vi "AutoLoadRoutines.vi"(1 "Reload Routines":bool, 2 "MotionPlanningNotifiers":T1, 3 "Auto Routines Storage Directory":path=path "/home/lvuser/AutoRoutines") -> (0 "Auto Routines":T2)   [LabVIEW 2017]
uses:
  TypeDef/AutoRoutines.ctl
  TypeDef/AutoRoutineSet.ctl
  TypeDefs/RobotComponents/MotionPlanningNotifiers.ctl
  PathPlannerSupport/TypeDefs/DrivePlanRequest.ctl
  TypeDef/AutoWaypointType.ctl
  Pathfinder/Pathfinder-LabVIEW/Pathfinder-Lib/VIs/Waypoint.ctl
  PathPlannerSupport/TypeDefs/DrivePlanResponse.ctl
  Pathfinder/Pathfinder-LabVIEW/Pathfinder-Lib/VIs/Segment.ctl
  Implements/Arm/TypeDefs/ArmPlanRequest.ctl
  Implements/Arm/TypeDefs/ArmTargetPosition.ctl
  Implements/Arm/TypeDefs/ArmPlanResponse.ctl
  General/MotionProfiling/TypeDefs/TrajectoryPoint.ctl
  <vilib>/Rock Robotics/WPI/ThirdParty/Phoenix-LabVIEW/Motor Controller/Controls/CTRE_Phoenix_MotorControl_TrajectoryPointTimeDur.ctl
  TypeDef/AutoStartingPositions.ctl
  TypeDef/AutoStep.ctl
  Implements/TypeDefs/IntakeState.ctl
  e61514f7-18c3-42f3-b2a8-fda8a5312ef7.vi
  55916f22-7f41-4e59-abc4-9fcd15d20e92.vi
  058e71e0-aaa7-4a66-86c1-b77b5f723853.vi
  <vilib>/Utility/file.llb/Read Delimited Spreadsheet (DBL).vi
  Pathfinder/Pathfinder-LabVIEW/Pathfinder-Lib/Pathfinder.lvlib
panel:
  in  "BackgroundFilePath":path=path "/home/lvuser/AutoPathImages/Background.png"
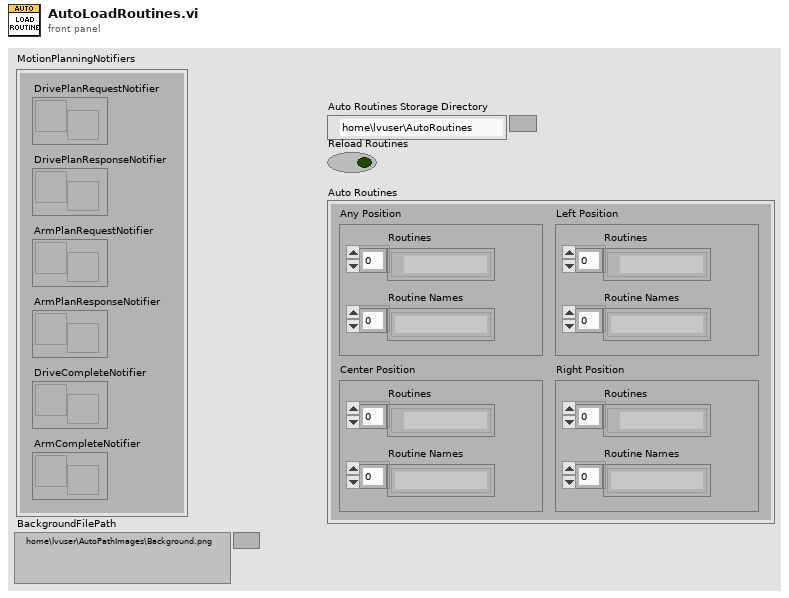
[diagram p1: front panel]
types:
  T1 = typedef "MotionPlanningNotifiers.ctl" = cluster{"DrivePlanRequestNotifier":refnum<notifier>, "DrivePlanResponseNotifier":refnum<notifier>, "ArmPlanRequestNotifier":refnum<notifier>, "ArmPlanResponseNotifier":refnum<notifier>, "DriveCompleteNotifier":refnum<notifier>, "ArmCompleteNotifier":refnum<notifier>}
  T2 = typedef "AutoRoutines.ctl" = cluster{"Any Position":T3, "Left Position":T3, "Center Position":T3, "Right Position":T3}
  T3 = typedef "AutoRoutineSet.ctl" = cluster{"Routine Names":string[], "Routines":path[]}
  T4 = typedef "AutoStartingPositions.ctl" = enum16{"Any", "Left", "Center", "Right"}
  T5 = typedef "ArmTargetPosition.ctl" = enum16{"Hold", "Switch", "Scale Low", "Scale High", "Climb", "Back Place"}
  T6 = typedef "IntakeState.ctl" = enum16{"Stop", "Forward", "Reverse", "Forward Open"}
  T7 = typedef "AutoWaypointType.ctl" = enum16{"Pathfinder Endpoint", "Pathfinder Waypoint", "Zero-Radius Turn Endpoint", "Stationary", "Vision Assist Endpoint", "Stop"}
  T8 = typedef "AutoStep.ctl" = cluster{"Waypoint Type":T7, "Waypoint":T9, "WaitTime (ms)":u16, "ArmPosition":T5, "IntakeState":T6, "Claw Open":bool, "ArmOffsetTime (ms)":u16, "ClawReleaseTime (ms)":i32}
  T9 = typedef "Pathfinder.lvlib/Waypoint.ctl" = cluster{"x":dbl, "y":dbl, "angle":dbl}
  T10 = typedef "AutoPreProcessedStep.ctl" = cluster{"DrivePath":T11, "ArmPath":T13, "Waypoint Type":T7, "WaitTime (ms)":u16, "ArmPosition":T5, "IntakeState":T6, "Claw Open":bool, "ArmOffsetTime (ms)":u16, "ClawReleaseTime (ms)":i32}
  T11 = typedef "DrivePlanResponse.ctl" = cluster{"LeftDriveTrajectory":T12[], "RightDriveTrajectory":T12[], "PlanTime (ms)":u32, "Execute":bool}
  T12 = typedef "Pathfinder.lvlib/Segment.ctl" = cluster{"dt":dbl, "x":dbl, "y":dbl, "position":dbl, "velocity":dbl, "acceleration":dbl, "jerk":dbl, "heading":dbl}
  T13 = typedef "ArmPlanResponse.ctl" = cluster{"RotateTrajectory":T14[], "ExtendTrajectory":T14[], "PlanTime (ms)":u32, "Execute":bool}
  T14 = typedef "TrajectoryPoint.ctl" = cluster{"Position ":dbl, "Velocity ":dbl, "Time (ms)":T15, "Last Point":bool}
  T15 = typedef "CTRE_Phoenix_MotorControl_TrajectoryPointTimeDur.ctl" = i32
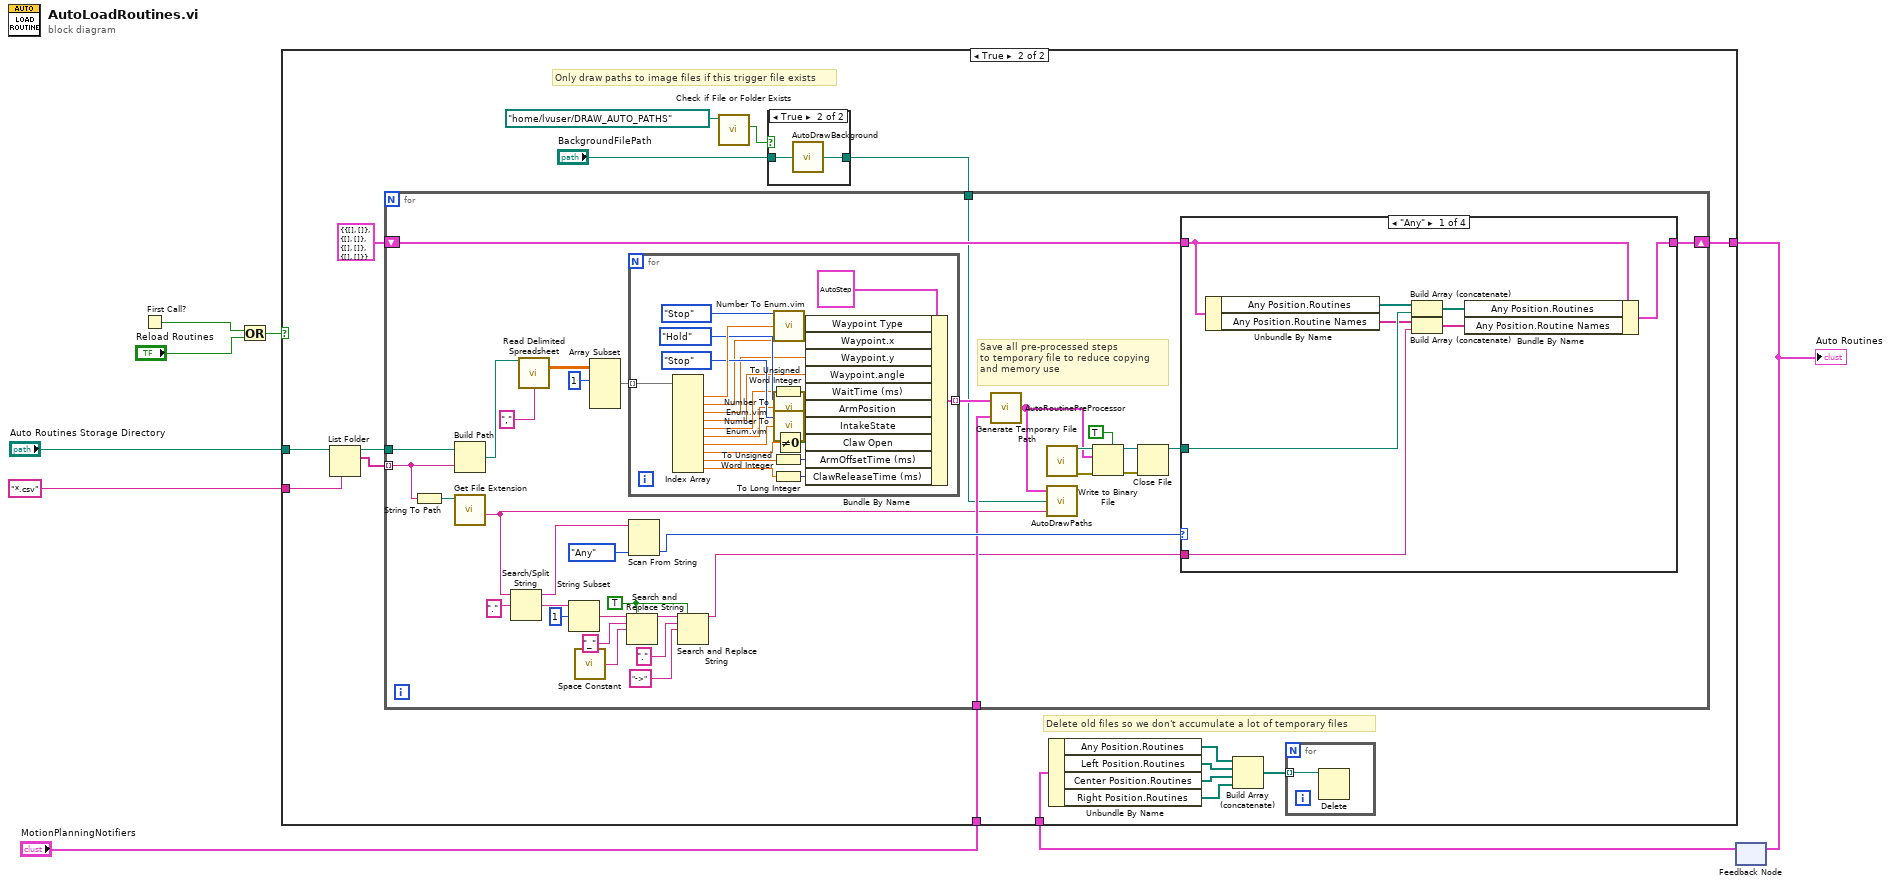
[diagram p0: block diagram]
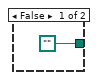
[diagram p3: hidden frame]
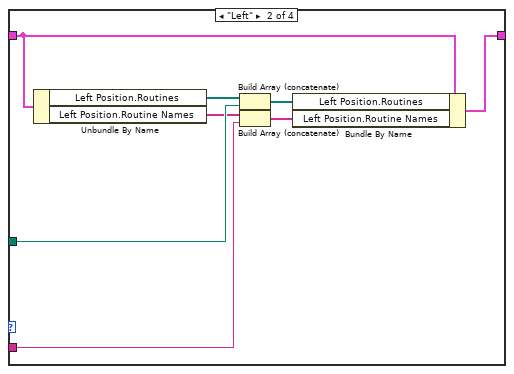
[diagram p4: hidden frame]
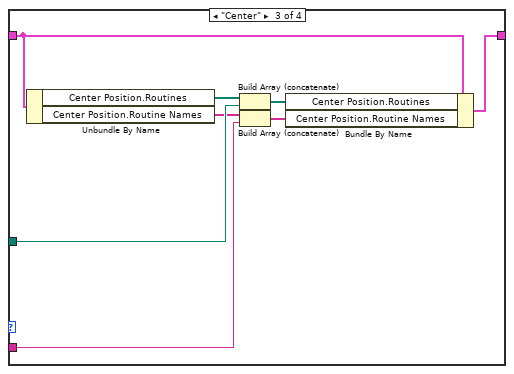
[diagram p5: hidden frame]
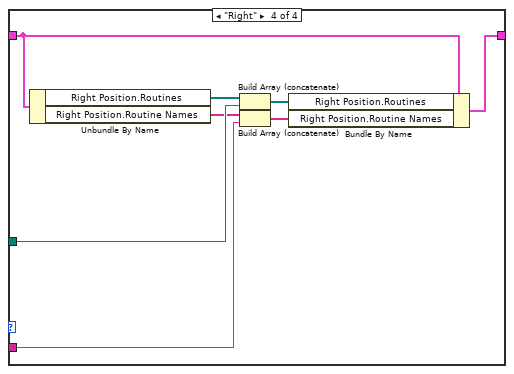
[diagram p6: hidden frame]
diagram:
  n1 = First Call?() -> (First Call?: T/F=w4:bool)
  n2 = Or(x=w4, y="Reload Routines") -> (x .or. y?=w6:bool)
  n3 = feedback #1() -> (w3:T2)  [unwired: 1 in]
  n4 = case shown="True" w6 {
    tunnel: "Auto Routines Storage Directory" -> [_ w26]
    tunnel: "*.csv" ("pattern") -> [_ w25]
    tunnel: [w9 w21] -> w2
    tunnel: w3 -> [w9 w19]
    tunnel: "MotionPlanningNotifiers" -> [_ w20]
    frame False {
    }
    frame True {
      # "Only draw paths to image files if this trigger file exists"
      # "Delete old files so we don't accumulate a lot of temporary files"
      n5 = List Folder(path=w26, pattern=w25) -> (path out=w24:path, filenames=w23:string[])  [unwired: 2 in, 2 out]
      n6 = call <vilib>:"Check if File or Folder Exists.vi"("path"=path "/home/lvuser/DRAW_AUTO_PATHS") -> ("file or folder exists?"=w11:bool)  [unwired: 8 in, 2 out]
      n7 = case shown="True" w11 {
        tunnel: "BackgroundFilePath" -> [_ w29]
        tunnel: [path "" w28] -> w12
        frame False {
        }
        frame True {
          n8 = call "AutoDrawBackground.vi"("File Path"=w29) -> ("File Path Out"=w28:path)
        }
      }
      n9 = for {
        tunnel: w24 -> [w62]
        tunnel: w23 -> [w43] mode=indexing
        shift-right: [w45] -> w21
        shift-left: T2 {"Any Position"={"Routine Names"=[], "Routines"=[]}, "Left Position"={"Routine Names"=[], "Routines"=[]}, "Center Position"={"Routine Names"=[], "Routines"=[]}, "Right Position"={"Routine Names"=[], "Routines"=[]}} ("Auto Routine") -> [w46]
        tunnel: w20 -> [w41]
        tunnel: w12 -> [w31]
        w53 = TRUE ("replace all? (F)")
        # "Save all pre-processed steps\nto temporary file to reduce copying\nand memory use"
        n10 = String To Path(string=w43) -> (path=w44:path)
        n11 = Build Path(base path=w62, name or relative path=w43) -> (appended path=w64:path)
        n12 = call <vilib>:"Get File Extension.vi"("file"=w44) -> ("filename without extension"=w32:string)  [unwired: 6 in, 4 out]
        n13 = Search/Split String(string=w32, search string/char (-)=".") -> (substring before match=w49:string, match + rest of string=w61:string)  [unwired: 1 in, 1 out]
        n14 = call-poly <vilib>:"Read Delimited Spreadsheet.vi"("file path (dialog if empty)"=w64, "delimiter (\\t)"="," ("delimiter (\\t)")) -> ("all rows"=w52:dbl[][])  [unwired: 8 in, 5 out]
        n15 = String Subset(string=w61, offset (0)=1) -> (substring=w59:string)  [unwired: 1 in]
        n16 = call <vilib>:"Space Constant.vi"() -> ("String"=w57:string)
        n17 = Array Subset(array=w52, index (row)=1 ("index")) -> (w50:dbl[][])  [unwired: 3 in]
        n18 = Search and Replace String(replace all?=w53, input string=w59, search string="_", replace string=w57) -> (result string=w56:string)  [unwired: 4 in, 3 out]
        n19 = for {
          tunnel: w50 -> [w120] mode=indexing
          tunnel: [w102] -> w42 mode=indexing
          n20 = Index Array(array=w120) -> (element #1=w115:dbl, element #2=w105:dbl, element #3=w104:dbl, element #4=w103:dbl, element #5=w107:dbl, element #6=w109:dbl, element #7=w110:dbl, element #8=w114:dbl, element #9=w101:dbl, element #10=w98:dbl)  [unwired: 10 in]
          n21 = To Unsigned Word Integer(number=w107) -> (unsigned 16bit integer=w106:u16)
          n22 = To Unsigned Word Integer(number=w101) -> (unsigned 16bit integer=w100:u16)
          n23 = To Long Integer(number=w98) -> (32bit integer=w99:i32)
          n24 = call "Number To Enum.vim"("number"=w115, "enum type"=AutoWaypointType."Stop" ("Waypoint Type")) -> ("number as enum"=w117:T7)
          n25 = call "Number To Enum.vim"("number"=w109, "enum type"=ArmTargetPosition."Hold" ("ArmPosition")) -> ("number as enum"=w111:T5)
          n26 = call "Number To Enum.vim"("number"=w110, "enum type"=IntakeState."Stop" ("IntakeState")) -> ("number as enum"=w113:T6)
          n27 = Not Equal To 0?(x=w114) -> (x != 0?=w118:bool)
          n28 = Bundle By Name(cluster=T8 {"Waypoint Type"=enum."Pathfinder Endpoint", "Waypoint"={"x"=0.0, "y"=0.0, "angle"=0.0}, "WaitTime (ms)"=0, "ArmPosition"=enum."Hold", "IntakeState"=enum."Stop", "Claw Open"=FALSE, "ArmOffsetTime (ms)"=0, "ClawReleaseTime (ms)"=0} ("Cluster"), "Waypoint Type"=w117, "Waypoint.x"=w105, "Waypoint.y"=w104, "Waypoint.angle"=w103, "WaitTime (ms)"=w106, "ArmPosition"=w111, "IntakeState"=w113, "Claw Open"=w118, "ArmOffsetTime (ms)"=w100, "ClawReleaseTime (ms)"=w99) -> (w102:T8)
        }
        n29 = Scan From String(input string=w49, default 1=AutoStartingPositions."Any" ("AutoStartingPosition")) -> (output 1=w47:T4)  [unwired: 3 in, 3 out]
        n30 = Search and Replace String(replace all?=w53, input string=w56, search string=".", replace string="->" ("replace string (\"\")")) -> (result string=w33:string)  [unwired: 4 in, 3 out]
        n31 = call "AutoRoutinePreProcessor.vi"("MotionPlanningNotifiers"=w41, "RawSteps"=w42) -> ("PreProcessedSteps"=w34:T10[])
        n32 = call <vilib>:"Generate Temporary File Path.vi"() -> ("error out"=w40:errorcluster, "Unique Temporary File Path"=w39:path)  [unwired: 10 in]
        n33 = call "AutoDrawPaths.vi"("RoutineName"=w32, "Background File Path"=w31, "RoutineSteps"=w34) -> ()  [unwired: 1 in]
        n34 = Write to Binary File(file (use dialog)=w39, data=w34, error in=w40, 5:TRUE ("prepend array or string size? (T)")) -> (refnum out=w38:refnum<file>, error out=w37:errorcluster)  [unwired: 2 in, 1 out]
        n35 = Close File(refnum=w38, error in=w37) -> (path=w36:path)  [unwired: 1 out]
        n36 = case shown="\"Any\"" w47 {
          tunnel: w33 -> [w69 w77 w85 w93]
          tunnel: w46 -> [w73 w81 w89 w97]
          tunnel: w36 -> [w71 w79 w87 w95]
          tunnel: [w66 w74 w82 w90] -> w45
          frame "Any" {
            n37 = Unbundle By Name(w73) -> ("Any Position.Routines"=w72:path[], "Any Position.Routine Names"=w70:string[])
            n38 = Build Array (concatenate)(w72, w71) -> (w67:path[])
            n39 = Build Array (concatenate)(w70, w69) -> (w68:string[])
            n40 = Bundle By Name(cluster=w73, "Any Position.Routines"=w67, "Any Position.Routine Names"=w68) -> (w66:T2)
          }
          frame "Left" {
            n41 = Unbundle By Name(w81) -> ("Left Position.Routines"=w80:path[], "Left Position.Routine Names"=w78:string[])
            n42 = Build Array (concatenate)(w80, w79) -> (w75:path[])
            n43 = Build Array (concatenate)(w78, w77) -> (w76:string[])
            n44 = Bundle By Name(cluster=w81, "Left Position.Routines"=w75, "Left Position.Routine Names"=w76) -> (w74:T2)
          }
          frame "Center" {
            n45 = Unbundle By Name(w89) -> ("Center Position.Routines"=w88:path[], "Center Position.Routine Names"=w86:string[])
            n46 = Build Array (concatenate)(w88, w87) -> (w83:path[])
            n47 = Build Array (concatenate)(w86, w85) -> (w84:string[])
            n48 = Bundle By Name(cluster=w89, "Center Position.Routines"=w83, "Center Position.Routine Names"=w84) -> (w82:T2)
          }
          frame "Right" {
            n49 = Unbundle By Name(w97) -> ("Right Position.Routines"=w96:path[], "Right Position.Routine Names"=w94:string[])
            n50 = Build Array (concatenate)(w96, w95) -> (w91:path[])
            n51 = Build Array (concatenate)(w94, w93) -> (w92:string[])
            n52 = Bundle By Name(cluster=w97, "Right Position.Routines"=w91, "Right Position.Routine Names"=w92) -> (w90:T2)
          }
        }
      }
      n53 = Unbundle By Name(w19) -> ("Any Position.Routines"=w18:path[], "Left Position.Routines"=w17:path[], "Center Position.Routines"=w16:path[], "Right Position.Routines"=w15:path[])
      n54 = Build Array (concatenate)(w18, w17, w16, w15) -> (w14:path[])
      n55 = for {
        tunnel: w14 -> [w30] mode=indexing
        n56 = Delete(path (use dialog)=w30) -> ()  [unwired: 4 in, 3 out]
      }
    }
  }
  "Auto Routines" <- w2
  n57 = feedback-in #1(w2) -> ()
